vi "RemoteVI Token Check.vi"(0 "query":string, 1 "token":string) -> (4 "ok?":bool)   [LabVIEW 2020, in "RemoteVI.lvlib"]
doc: "Checks the share's access token (docs\\security.md): query is the request target after the path, with or without its leading question mark; every question mark counts as a parameter separator like an ampersand. The first t parameter is compared with token in constant time (the bytes are XORed and the differences ORed up, no early exit); ok? is TRUE only when both have the same length, token is not empty (fail closed) and every byte matches. The value is compared as sent, without percent-decoding (tokens are hex). Pure function, cannot fail. Reference: tokenOk() in tools\\lib\\http.mjs, vectors tests\\vectors\\http.json (tokens)."
uses:
  RemoteVI.lvlib
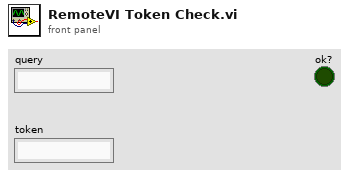
[diagram p1: front panel]
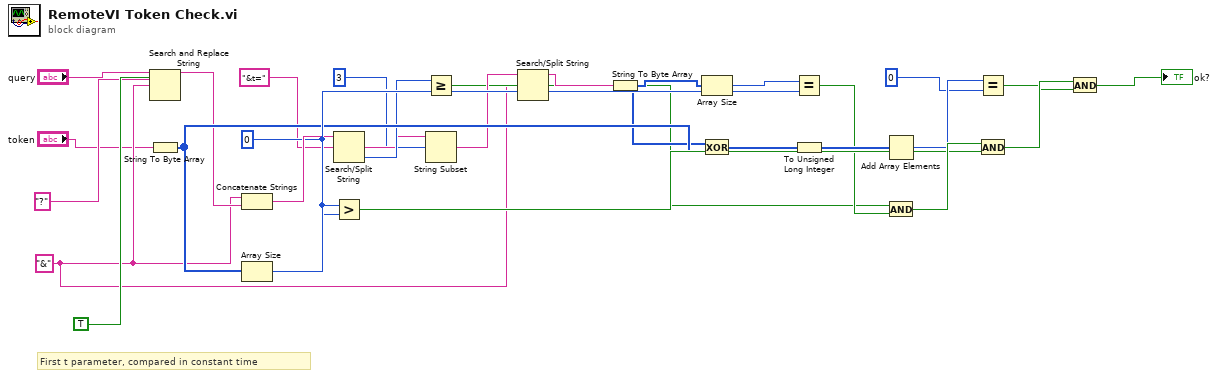
[diagram p0: block diagram]
diagram:
  w8 = 0
  w4 = "&"
  # "First t parameter, compared in constant time"
  n1 = Search and Replace String(replace all?=TRUE, input string="query", search string="?", replace string=w4) -> (result string=w10:string)  [unwired: 4 in, 3 out]
  n2 = String To Byte Array(string="token") -> (unsigned byte array=w18:u8[])
  n3 = Concatenate Strings(w4, w10) -> (w11:string)
  n4 = Array Size(array=w18) -> (size(s)=w20:i32)
  n5 = Search/Split String(string=w11, search string/char (-)="&t=") -> (match + rest of string=w12:string, offset of match=w13:i32)  [unwired: 1 in, 1 out]
  n6 = Greater?(x=w20, y=w8) -> (0:w22:bool)
  n7 = Greater Or Equal?(x=w13, y=w8) -> (x >= y?=w14:bool)
  n8 = String Subset(string=w12, offset (0)=3) -> (substring=w15:string)  [unwired: 1 in]
  n9 = Search/Split String(string=w15, search string/char (-)=w4) -> (substring before match=w16:string)  [unwired: 1 in, 2 out]
  n10 = String To Byte Array(string=w16) -> (unsigned byte array=w17:u8[])
  n11 = Array Size(array=w17) -> (size(s)=w19:i32)
  n12 = Exclusive Or(1:w18, 2:w17) -> (0:w23:u8[])
  n13 = Equal?(x=w19, y=w20) -> (x = y?=w21:bool)
  n14 = To Unsigned Long Integer(number=w23) -> (unsigned 32bit integer=w24:u32[])
  n15 = Add Array Elements(numeric array=w24) -> (sum=w25:u32)
  n16 = And(x=w14, y=w21) -> (x .and. y?=w27:bool)
  n17 = Equal?(x=w25, y=u32 0) -> (x = y?=w26:bool)
  n18 = And(x=w27, y=w22) -> (x .and. y?=w28:bool)
  n19 = And(x=w28, y=w26) -> (x .and. y?=→"ok?":bool)
